vi "CSM - Sync Configuration Variables to File.vi"(4 "Write UnSupported Datatype?(F)":bool, 5 "All Temp Variable to Default Ini(F)":bool, 8 "error in (no error)":errorcluster) -> (2 "error out":errorcluster)   [LabVIEW 2017, in "INI-Static-Variable-Support.lvlib"]
doc: "Synchronizes variables in memory to the specified configuration file.\n\n<b>Note</b>: Only permanent variables are synchronized to the file. If you want to write temporary variables to the file, you need to mark the temporary variables as permanent in advance.\n\n\n> [!NOTE] <b>CSM INI-Variable Configuration File Path</b>\n>\n> - <b>Development State</b>: The first INI configuration file found in the Application Directory. If no configuration file exists, it defaults to `csm-app.ini`.\n> - <b>Post-Compilation</b>: An INI configuration file in the same directory as the executable file, with the same name as the executable. LabVIEW automatically generates this file after compilation.\n> - Supports loading multiple configuration files. Configuration items in files loaded later will overwrite identical items in previously loaded files.\n> - Configuration files can use the `[__include]` section to reference other configuration files.\n> - Supports both relative and absolute paths.\n> - Relative paths are relative to the path of the current configuration file.\n> - The name of the configuration file in the `[__include]` section is not critical, as long as the path is correct.\n> - To avoid circular references, the same configuration file will be automatically ignored if loaded a second time.\n\n\n-- <b>Controls</b> --\n- <b>All Temp Variable to Default Ini(F)</b>: Whether to synchronize all temporary variables to the default INI file.\n- <b>Write UnSupported Datatype?(F)</b>: Whether to write unsupported data types."
uses:
  INI-Static-Variable-Support.lvlib
  _Support/_fgv-oper.ctl
  <userlib>/_NEVSTOP/Communicable State Machine(CSM)/_Support/ChangeFlag/ChangeFlag-Read.vi
  <userlib>/_NEVSTOP/Communicable State Machine(CSM)/_Support/ChangeFlag/ChangeFlagDB.vi
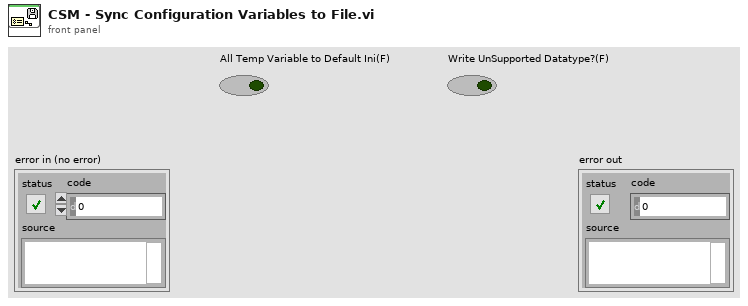
[diagram p1: front panel]
types:
  T1 = typedef "INI-Static-Variable-Support.lvlib/_fgv-oper.ctl" = enum16{"Read", "Write", "Sync", "Sessions", "List Keys", "Load", "List Files", "List Variables", "List Permanent Variables", "Mark Temp Variable as Permenent", "unload", "INIConfig(Memory)", "Reset", "Restore Variable Value"}
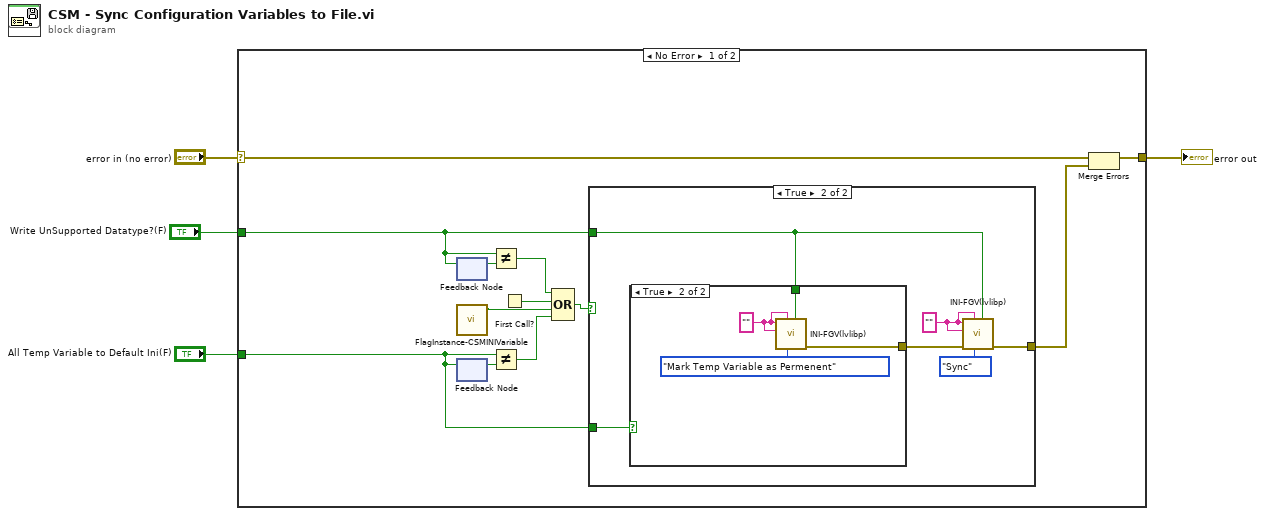
[diagram p0: block diagram]
diagram:
  n1 = case shown="No Error" "error in (no error)" {
    selector: "error in (no error)" -> [w15 w27]
    tunnel: [w16 w27] -> w4
    tunnel: "All Temp Variable to Default Ini(F)" -> [w9 _]
    tunnel: "Write UnSupported Datatype?(F)" -> [w7 _]
    frame No Error {
      n2 = feedback #1() -> (w8:bool)  [unwired: 1 in]
      n3 = feedback-in #1(w7) -> ()
      n4 = call "FlagInstance-CSMINIVariable.vi"() -> ("Changed"=w5:bool)  [unwired: 10 in, 1 out]
      n5 = feedback #2() -> (w11:bool)  [unwired: 1 in]
      n6 = feedback-in #2(w9) -> ()
      n7 = Not Equal?(x=w7, y=w8) -> (x != y?=w6:bool)
      n8 = Not Equal?(x=w9, y=w11) -> (x != y?=w10:bool)
      n9 = First Call?() -> (First Call?: T/F=w14:bool)
      n10 = Compound Arithmetic op=OR(w6, w14, w5, w10) -> (w13:bool)
      n11 = case shown="True" w13 {
        tunnel: [_ w21] -> w12
        tunnel: w9 -> [_ w19]
        tunnel: w7 -> [_ w18]
        frame False {
        }
        frame True {
          w17 = "" (">> Variable Name >>")
          n12 = case shown="True" w19 {
            tunnel: [_ w25] -> w20
            tunnel: w18 -> [_ w24]
            frame False {
            }
            frame True {
              w23 = "" (">> Variable Name >>")
              n13 = call "INI-FGV(lvlibp).vi"("Write If not found?"=w24, "Enum"=_fgv-oper."Mark Temp Variable as Permenent", "Prefered Section"=w23, ">> Default Value >>"=w23, ">> Variable Name >>"=w23) -> ("error out"=w25:errorcluster)  [unwired: 3 in, 3 out]
            }
          }
          n14 = call "INI-FGV(lvlibp).vi"("Write If not found?"=w18, "Enum"=_fgv-oper."Sync", "Prefered Section"=w17, "error IN"=w20, ">> Default Value >>"=w17, ">> Variable Name >>"=w17) -> ("error out"=w21:errorcluster)  [unwired: 2 in, 3 out]
        }
      }
      n15 = Merge Errors(w15, w12) -> (w16:errorcluster)
    }
    frame Error {
    }
  }
  "error out" <- w4
